vi "Chart Data.vi"(6 "Set Time":bool, 8 "error in (no error)":errorcluster, 9 "End":dbl, 10 "Start":dbl, 11 "HistorianCharting in":refnum<class "HistorianCharting.lvclass">) -> (0 "error out":errorcluster, 3 "HistorianCharting out":refnum<class "HistorianCharting.lvclass">)   [LabVIEW 2020, in "VolatusGUIElements.lvlib" / "HistorianCharting.lvclass"]
uses:
  HistorianCharting.lvclass
  Decimation Params.ctl
  HistorianCharting.lvclass/HistorianCharting.ctl
  Plot Time Range.vi
  Pixel Segments.vi
  Decimate Segments.vi
  First Last Samples.vi
  VolatusHistorian/Group Buffer DBL/Group Buffer DBL.lvclass
  VolatusGUIElements.lvlib
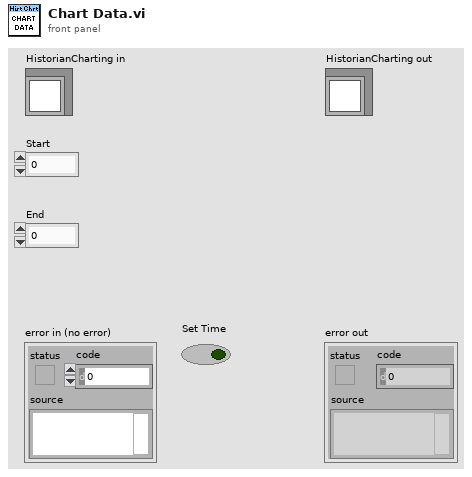
[diagram p1: front panel]
types:
  T1 = typedef "VolatusGUIElements.lvlib/Decimation Params.ctl" = cluster{"Width":i32, "Start":dbl, "End":dbl}
  T2 = typedef "VolatusGUI.lvlib/Historian Charting Manager.lvclass/X-Axis Type.ctl" = enum16{"Time", "Channel"}
  T3 = typedef "VolatusGUIElements.lvlib/HistorianCharting.lvclass/Buffer Info.ctl" = cluster{"Buffer":refnum<class "Group Buffer DBL.lvclass">, "Channels":string[], "Plot Indices":i32[]}
  T4 = typedef "VolatusHistorian.lvlib/Group Data.ctl" = cluster{"Name":string, "Timestamp":dbl[], "Channels":T5[]}
  T5 = typedef "VolatusHistorian.lvlib/Channel Data.ctl" = cluster{"Name":string, "Data":dbl[]}
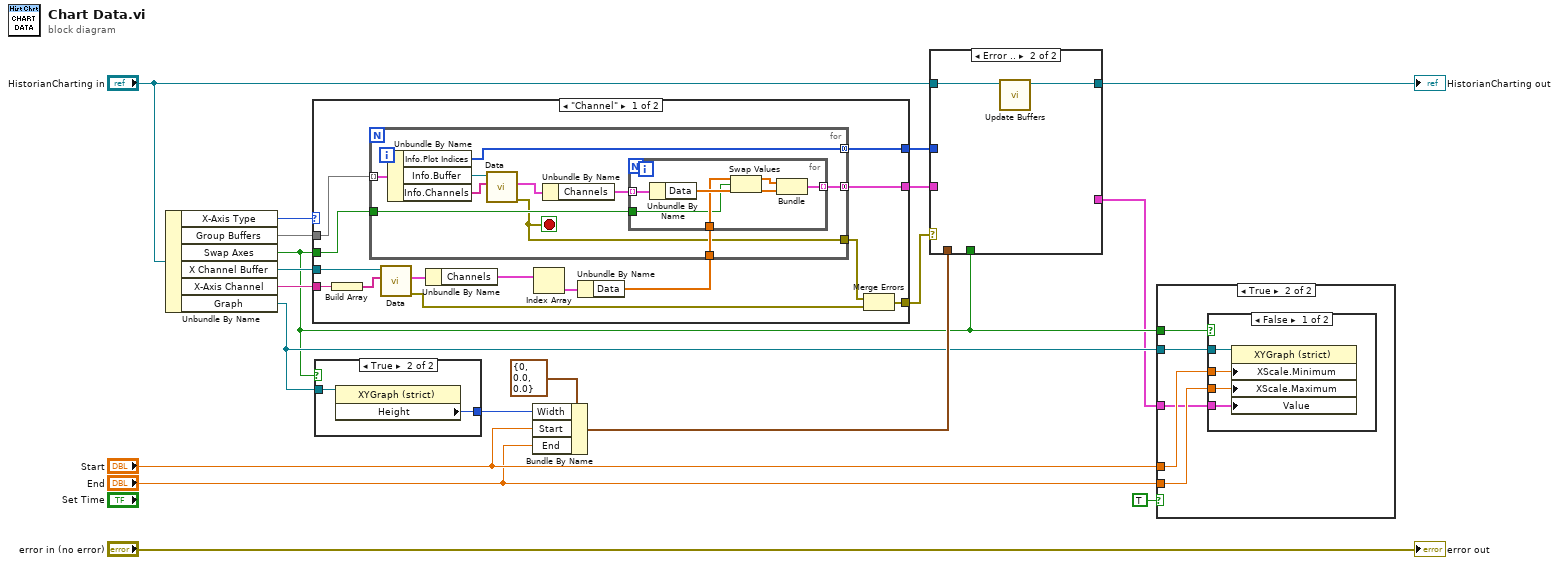
[diagram p0: block diagram]
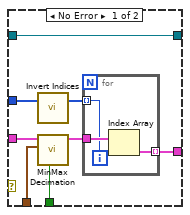
[diagram p2: hidden frame]
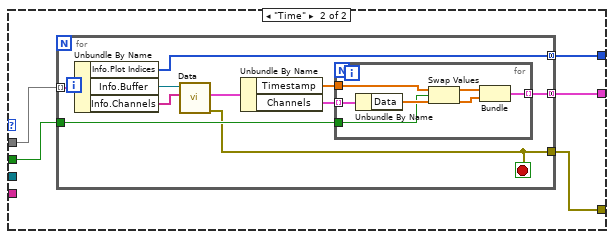
[diagram p3: hidden frame]
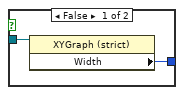
[diagram p4: hidden frame]
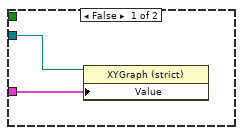
[diagram p5: hidden frame]
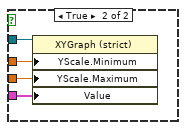
[diagram p6: hidden frame]
diagram:
  n1 = Unbundle By Name("HistorianCharting in") -> ("X-Axis Type"=w17:T2, "Group Buffers"=w18:map{string, T3}, "Swap Axes"=w7:bool, "X Channel Buffer"=w16:refnum<class "Group Buffer DBL.lvclass">, "X-Axis Channel"=w15:string, "Graph"=w10:refnum<vi>)
  n2 = case shown="\"Channel\"" w17 {
    tunnel: w18 -> [w30 w55]
    tunnel: w7 -> [w29 w54]
    tunnel: w16 -> [w32 _]
    tunnel: w15 -> [w33 _]
    tunnel: [w24 w53] -> w14
    tunnel: [w23 w52] -> w6
    tunnel: [w20 w51] -> w3
    frame "Channel" {
      n3 = Build Array(w33) -> (w31:string[])
      n4 = call "Data.vi"("Channels (All)"=w31, "Group Buffer DBL in"=w32) -> ("error out"=w22:errorcluster, "Group Data"=w28:T4)  [unwired: 7 in, 1 out]
      n5 = Unbundle By Name(w28) -> ("Channels"=w27:T5[])
      n6 = Index Array(array=w27) -> (element=w26:T5)  [unwired: 1 in]
      n7 = Unbundle By Name(w26) -> ("Data"=w25:dbl[])
      n8 = for {
        tunnel: w30 -> [w43] mode=indexing
        tunnel: w29 -> [w38]
        tunnel: [w37] -> w24 mode=concatenating
        tunnel: [w36] -> w23 mode=concatenating
        tunnel: w25 -> [w35]
        tunnel: [w34] -> w21
        stop <- w34 stop-if-true
        n9 = Unbundle By Name(w43) -> ("Info.Plot Indices"=w36:i32[], "Info.Buffer"=w42:refnum<class "Group Buffer DBL.lvclass">, "Info.Channels"=w41:string[])
        n10 = call "Data.vi"("Channels (All)"=w41, "Group Buffer DBL in"=w42) -> ("error out"=w34:errorcluster, "Group Data"=w40:T4)  [unwired: 7 in, 1 out]
        n11 = Unbundle By Name(w40) -> ("Channels"=w39:T5[])
        n12 = for {
          tunnel: w39 -> [w50] mode=indexing
          tunnel: w38 -> [w44]
          tunnel: [w49] -> w37 mode=indexing
          tunnel: w35 -> [w45]
          n13 = Unbundle By Name(w50) -> ("Data"=w46:dbl[])
          n14 = Swap Values(12:w45, 13:w44, 14:w46) -> (1:w48:dbl[], 3:w47:dbl[])
          n15 = Bundle(w48, w47) -> (w49:cluster{dbl[], dbl[]})  [unwired: 1 in]
        }
      }
      n16 = Merge Errors(w21, w22) -> (w20:errorcluster)
    }
    frame "Time" {
      n17 = for {
        tunnel: w55 -> [w65] mode=indexing
        tunnel: w54 -> [w59]
        tunnel: [w58] -> w53 mode=concatenating
        tunnel: [w57] -> w52 mode=concatenating
        tunnel: [w56] -> w51
        stop <- w56 stop-if-true
        n18 = Unbundle By Name(w65) -> ("Info.Plot Indices"=w57:i32[], "Info.Buffer"=w64:refnum<class "Group Buffer DBL.lvclass">, "Info.Channels"=w63:string[])
        n19 = call "Data.vi"("Channels (All)"=w63, "Group Buffer DBL in"=w64) -> ("error out"=w56:errorcluster, "Group Data"=w62:T4)  [unwired: 7 in, 1 out]
        n20 = Unbundle By Name(w62) -> ("Timestamp"=w61:dbl[], "Channels"=w60:T5[])
        n21 = for {
          tunnel: w61 -> [w66]
          tunnel: w60 -> [w72] mode=indexing
          tunnel: w59 -> [w69]
          tunnel: [w71] -> w58 mode=indexing
          n22 = Unbundle By Name(w72) -> ("Data"=w70:dbl[])
          n23 = Swap Values(12:w66, 13:w69, 14:w70) -> (1:w67:dbl[], 3:w68:dbl[])
          n24 = Bundle(w67, w68) -> (w71:cluster{dbl[], dbl[]})  [unwired: 1 in]
        }
      }
    }
  }
  n25 = case shown="True" w7 {
    tunnel: w10 -> [w74 w76]
    tunnel: [w73 w75] -> w11
    frame False {
      n26 = property class="XYGraph (strict)"(reference=w74) -> ("Width"=w73:u32)  [unwired: 1 in, 2 out]
    }
    frame True {
      n27 = property class="XYGraph (strict)"(reference=w76) -> ("Height"=w75:u32)  [unwired: 1 in, 2 out]
    }
  }
  n28 = Bundle By Name(cluster=T1 {"Width"=0, "Start"=0.0, "End"=0.0} ("Params"), "Width"=w11, "Start"="Start", "End"="End") -> (w12:T1)
  n29 = case shown="Error .." w3 {
    tunnel: w14 -> [w84 _]
    tunnel: w12 -> [w83 _]
    tunnel: w7 -> [w82 _]
    tunnel: w6 -> [w80 _]
    tunnel: [w78 _] -> w5
    tunnel: "HistorianCharting in" -> [w77 w89]
    tunnel: [w77 w88] -> w1
    frame No Error {
      n30 = call "Invert Indices.vi"("Destination Indices"=w80) -> ("Source Indices"=w79:i32[])  [unwired: 6 in]
      n31 = call "MinMax Decimation.vi"("Swap Axes (F)"=w82, "Params"=w83, "XY Data"=w84) -> ("MinMax Data"=w81:cluster{dbl[], dbl[]}[])  [unwired: 8 in]
      n32 = for {
        tunnel: w81 -> [w87]
        tunnel: w79 -> [w86] mode=indexing
        tunnel: [w85] -> w78 mode=indexing
        n33 = Index Array(array=w87, index=w86) -> (element=w85:cluster{dbl[], dbl[]})
      }
    }
    frame Error {
      n34 = call "Update Buffers.vi"("HistorianCharting in"=w89) -> ("HistorianCharting out"=w88:refnum<class "HistorianCharting.lvclass">)  [unwired: 9 in, 1 out]
    }
  }
  "HistorianCharting out" <- w1
  n35 = case shown="True" TRUE {
    tunnel: w10 -> [w91 w96]
    tunnel: w5 -> [w90 w93]
    tunnel: "Start" -> [_ w95]
    tunnel: "End" -> [_ w94]
    tunnel: w7 -> [_ w92]
    frame False {
      n36 = property class="XYGraph (strict)"(reference=w91, "Value"=w90) -> ()  [unwired: 1 in, 2 out]
    }
    frame True {
      n37 = case shown="False" w92 {
        tunnel: w96 -> [w100 w104]
        tunnel: w95 -> [w99 w103]
        tunnel: w94 -> [w98 w102]
        tunnel: w93 -> [w97 w101]
        frame False {
          n38 = property class="XYGraph (strict)"(reference=w100, "XScale.Minimum"=w99, "XScale.Maximum"=w98, "Value"=w97) -> ()  [unwired: 1 in, 2 out]
        }
        frame True {
          n39 = property class="XYGraph (strict)"(reference=w104, "YScale.Minimum"=w103, "YScale.Maximum"=w102, "Value"=w101) -> ()  [unwired: 1 in, 2 out]
        }
      }
    }
  }
  "error out" <- "error in (no error)"
